vi "var to string (int).vi"(10 "Numeric type":i32, 11 "reference":refnum<vi>) -> (3 "decimal integer string":string)   [LabVIEW 2025]
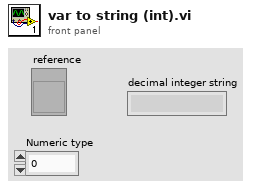
[diagram p1: front panel]
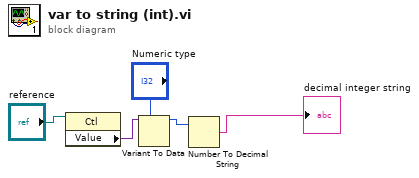
[diagram p0: block diagram]
diagram:
  n1 = property class="Ctl"(reference="reference") -> ("Value"=w5:variant)  [unwired: 1 in, 2 out]
  n2 = Variant To Data(type="Numeric type", Variant=w5) -> (data=w3:i32)  [unwired: 1 in, 1 out]
  n3 = Number To Decimal String(number=w3) -> (decimal integer string=→"decimal integer string":string)  [unwired: 1 in]
